vi "Get Drive Current.vi"(8 "Motors In":T1 {"Steer Scaling" format="%.2f"; "Drive Scaling" format="%.2f"; "Pod Locations (ft)"."Right Back Position" format="%.2f"; "Pod Locations (ft)"."Right Front Position" format="%.2f"; "Pod Locations (ft)"."Left Back Position" format="%.2f"; "Pod Locations (ft)"."Left Front Position" format="%.2f"}) -> (0 "Motors Out":T1 {"Steer Scaling" format="%.2f"; "Drive Scaling" format="%.2f"; "Pod Locations (ft)"."Right Back Position" format="%.2f"; "Pod Locations (ft)"."Right Front Position" format="%.2f"; "Pod Locations (ft)"."Left Back Position" format="%.2f"; "Pod Locations (ft)"."Left Front Position" format="%.2f"})   [LabVIEW 2023]
uses:
  swerve-template/Type Definitions/Hardware/Swerve Drives/(NEO-NEO-ThroughBore-Pigeon2) Swerve.ctl
  <vilib>/REV Custom Controls/REVSparkRefnum.ctl
  swerve-template/Type Definitions/Data/Pod Positions.ctl
  <resource>/objmgr/REVSpark.rc
  <vilib>/REVLibDriver/REVLibDriver.lvlib
panel:
  out "total current":sgl
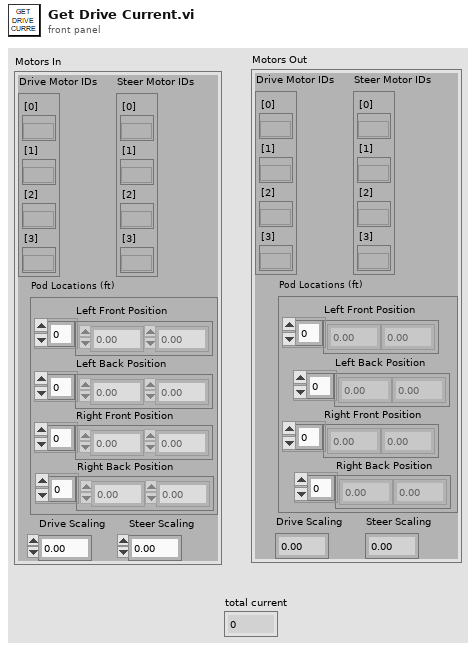
[diagram p1: front panel]
types:
  T1 = typedef "(NEO-NEO-ThroughBore-Pigeon2) Swerve.ctl" = cluster{"Drive Motor IDs":cluster{"[0]":T2, "[1]":T2, "[2]":T2, "[3]":T2}, "Steer Motor IDs":cluster{"[0]":T2, "[1]":T2, "[2]":T2, "[3]":T2}, "Pod Locations (ft)":T3, "Drive Scaling":dbl, "Steer Scaling":dbl}
  T2 = typedef "REVLibDriver.lvlib/REVSparkRefnum.ctl" = refnum<k20>
  T3 = typedef "Pod Positions.ctl" = cluster{"Left Front Position":dbl[], "Left Back Position":dbl[], "Right Front Position":dbl[], "Right Back Position":dbl[]}
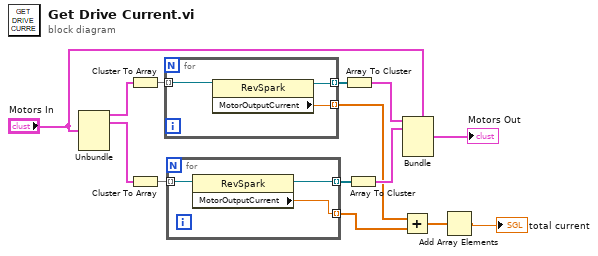
[diagram p0: block diagram]
diagram:
  n1 = Unbundle("Motors In") -> ("Drive Motor IDs"=w14:cluster{"[0]":T2, "[1]":T2, "[2]":T2, "[3]":T2}, "Steer Motor IDs"=w13:cluster{"[0]":T2, "[1]":T2, "[2]":T2, "[3]":T2})  [unwired: 3 out]
  n2 = Cluster To Array(cluster=w14) -> (array=w12:T2[])
  n3 = Cluster To Array(cluster=w13) -> (array=w11:T2[])
  n4 = for {
    tunnel: w12 -> [w15] mode=indexing
    tunnel: [w17] -> w9 mode=indexing
    tunnel: [w16] -> w4 mode=indexing
    n5 = property class="RevSpark"(reference=w15) -> (reference out=w17:T2, "MotorOutputCurrent"=w16:sgl)  [unwired: 1 in, 1 out]
  }
  n6 = for {
    tunnel: w11 -> [w20] mode=indexing
    tunnel: [w18] -> w7 mode=indexing
    tunnel: [w19] -> w3 mode=indexing
    n7 = property class="RevSpark"(reference=w20) -> (reference out=w18:T2, "MotorOutputCurrent"=w19:sgl)  [unwired: 1 in, 1 out]
  }
  n8 = Array To Cluster(array=w9) -> (cluster=w8:cluster{"[0]":T2, "[1]":T2, "[2]":T2, "[3]":T2})
  n9 = Array To Cluster(array=w7) -> (cluster=w6:cluster{"[0]":T2, "[1]":T2, "[2]":T2, "[3]":T2})
  n10 = Add(x=w4, y=w3) -> (x+y=w2:sgl[])
  n11 = Bundle(cluster="Motors In", "Drive Motor IDs"=w8, "Steer Motor IDs"=w6) -> (→"Motors Out":T1)  [unwired: 3 in]
  n12 = Add Array Elements(numeric array=w2) -> (sum=→"total current":sgl)
